vi "Apply ROIs.vi"(5 "Function":T1=enum."Write-from dataset", 7 "Mode (Redraw All)":T2, 8 "error in (no error)":errorcluster, 9 "ROIs Info []":T3[](array[typedef]) {"FOV" min=1.0 max=10.0 step=1.0; "Frame Size" min=1.0 max=10.0 step=1.0; "Laser Power" min=1.0 max=10.0 step=0.10000000149011612; "Rel. Resolution" min=1.0 max=10.0 step=1.0; "POI Dwell time" min=1.0 max=10.0 step=0.10000000149011612; "Zoom" min=1.0 max=10.0 step=0.10000000149011612}) -> (0 "error out":errorcluster, 1 "Number of ROI":i32, 3 "No ROI":bool)   [LabVIEW 2020]
uses:
  Typedefs/ROI spec.ctl
  Typedefs/ROI ID Enum.ctl
  ROI Entry screen/Typedefs/Redraw ROI.ctl
  Typedefs/ROI management FG states.ctl
  ROI Entry screen/Typedefs/FGV ROI Time Ops.ctl
  Typedefs/ROI management Input cluster.ctl
  Global Variables/General Globals.vi
  <resource>/objmgr/IMAQImage.rc
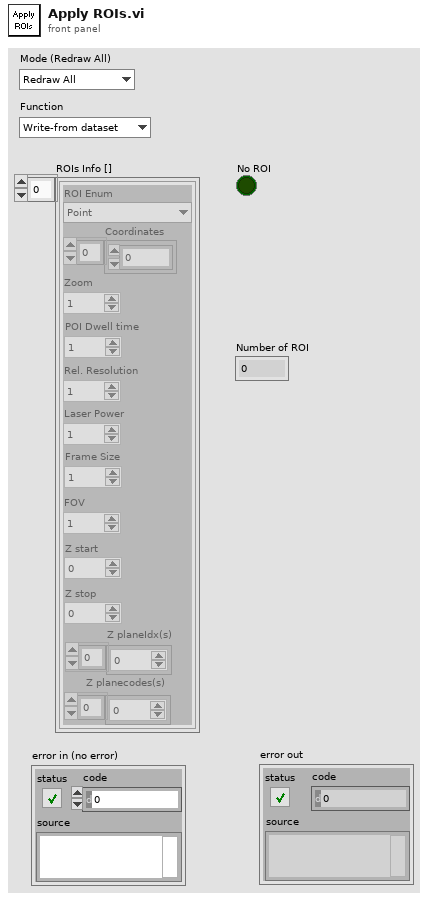
[diagram p1: front panel]
types:
  T1 = typedef "ROI management FG states.ctl" = enum16{"Read", "Write", "Write-from dataset", "Clear Last", "Clear All", "Delete ROI", "Update ROIs time", "Reload last ROI set", "Modify ROI Parameters", "Offset all ROI", "Offset visible ROI", "Modify Dwell Time", "Modify Laser Power"}
  T2 = typedef "Redraw ROI.ctl" = enum16{"Redraw All", "Redraw Deselected", "Draw Last", "Redraw Selected"}
  T3 = typedef "ROI spec.ctl" = cluster{"ROI Enum":T4, "Coordinates":i32[], "Zoom":dbl, "POI Dwell time":dbl, "Rel. Resolution":dbl, "Laser Power":dbl, "Frame Size":dbl, "FOV":dbl, "Z start":dbl, "Z stop":dbl, "Z planeIdx(s)":i32[], "Z planecodes(s)":u8[]}
  T4 = typedef "ROI ID Enum.ctl" = enum16{"Point", "MiniScan", "Comp. MiniScan", "Rectangle", "Comp. volume", "Arb. plane point", "None"}
  T5 = typedef "ROI parameters data type.ctl" = cluster{"ROI index":dbl, "ROI ID":dbl, "ROI Time (ns)":dbl, "Pixels in ROI":dbl, "X start":dbl, "Y start":dbl, "Z start":dbl, "X stop":dbl, "Y stop":dbl, "Z stop":dbl, "Angle (deg)":dbl, "Composite ID":dbl, "Number of lines":dbl, "Frame Size":dbl, "Zoom":dbl, "Laser Power (%)":dbl, "ROI group ID":dbl, "Resolution":dbl, "Dwell Time per pixel":dbl, "Pixels per miniscan":dbl, "Original FOV (um)":dbl, "Apparent Frame Size":dbl, "Z Plane Idx":i32[], "Z Plane codes":i32[]}
  T6 = typedef "FGV ROI Time Ops.ctl" = enum16{"Read", "Write Cycle Time", "Write Cycle Rate"}
  T7 = typedef "ROI management Input cluster.ctl" = cluster{"ROI Type":T4, "XY Coordinates":i32[], "Motor Z Planes":dbl[], "Dwell time per POI or per pixel (us)":dbl, "Frame size":i32, "Zoom":dbl, "Rel. Resolution":dbl, "FOV":dbl, "Laser Power (%)":dbl, "Z Plane codes":u8[], "Z start":dbl, "Z stop":dbl, "Z Plane Idx(s)":i32[]}
  T8 = typedef "IMAQ Image.ctl" = refnum<image>
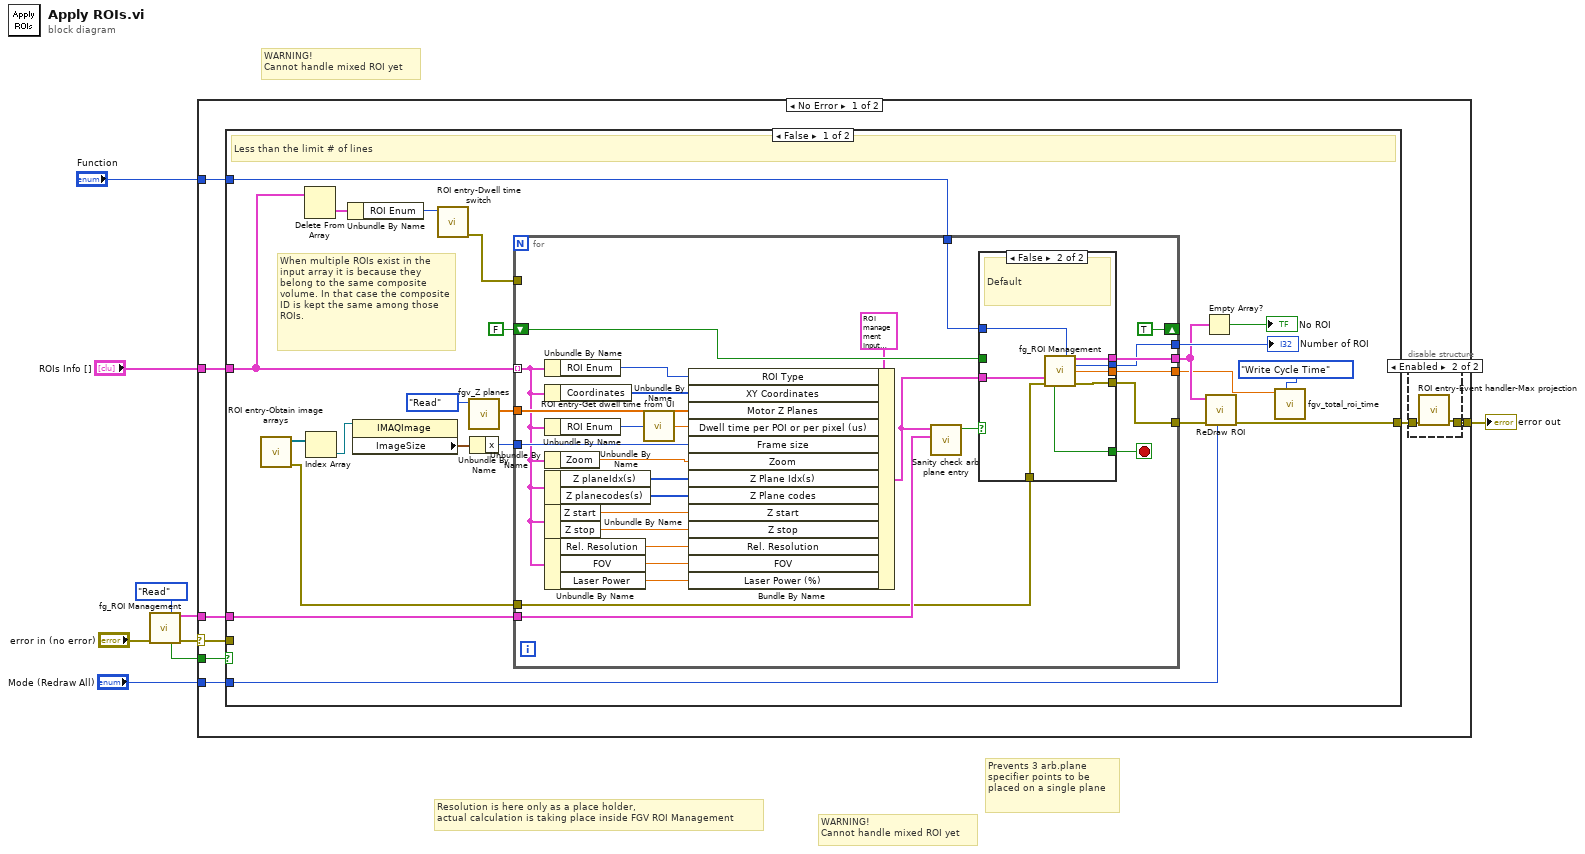
[diagram p0: block diagram]
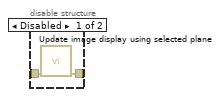
[diagram p2: hidden frame]
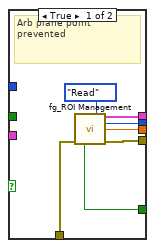
[diagram p3: hidden frame]
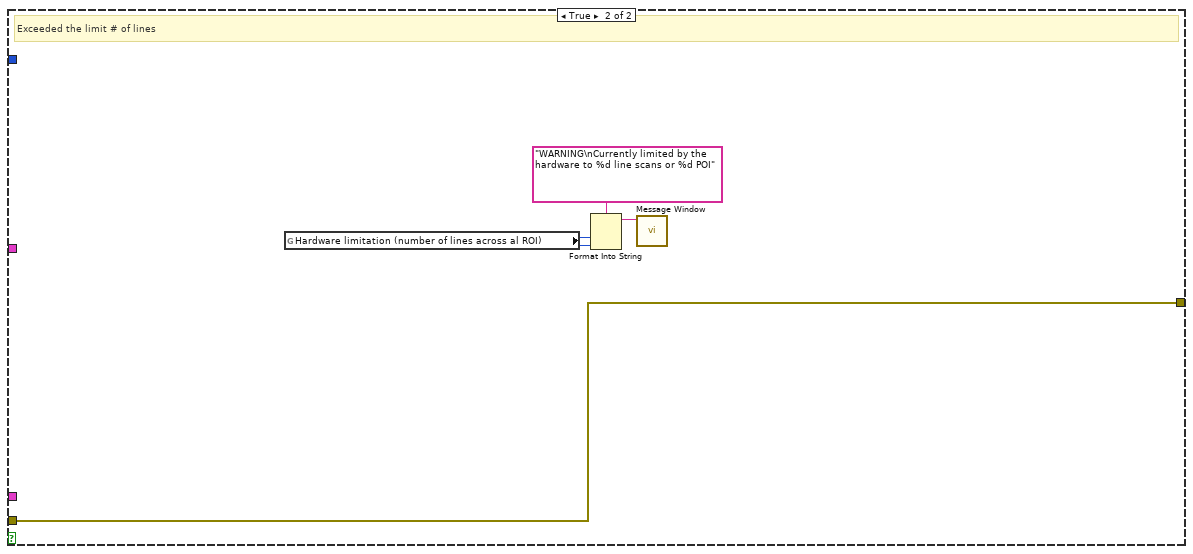
[diagram p4: hidden frame]
diagram:
  # "Resolution is here only as a place holder,\nactual calculation is taking place inside FGV ROI Management"
  # "WARNING!\nCannot handle mixed ROI yet"
  # "WARNING!\nCannot handle mixed ROI yet"
  # "Prevents 3 arb.plane specifier points to be placed on a single plane"
  n1 = call "fg_ROI Management.vi"("Function"=ROI_management_FG_states."Read", "error in (no error)"="error in (no error)") -> ("ROI Setup"=w6:T5[], "No lines left"=w1:bool, "error out"=w5:errorcluster)  [unwired: 7 in, 4 out]
  n2 = case shown="No Error" w5 {
    selector: w5 -> [w15 w91]
    tunnel: w6 -> [w17 _]
    tunnel: [w13 w91] -> w4
    tunnel: "ROIs Info []" -> [w16 _]
    tunnel: "Mode (Redraw All)" -> [w12 _]
    tunnel: "Function" -> [w11 _]
    tunnel: w1 -> [w10 _]
    frame No Error {
      n3 = case shown="False" w10 {
        tunnel: w17 -> [w38 _]
        tunnel: w16 -> [w28 _]
        tunnel: [w34 w90] -> w14
        tunnel: w15 -> [_ w90]
        tunnel: w12 -> [w29 _]
        tunnel: w11 -> [w24 _]
        frame False {
          # "When multiple ROIs exist in the input array it is because they belong to the same composite volume. In that case the composite ID is kept the same among those ROIs."
          # "Less than the limit # of lines"
          n4 = call "ROI entry-Obtain image arrays.vi"() -> ("error IO"=w33:errorcluster, "RedImageArray"=w37:T8[])  [unwired: 10 in]
          n5 = Delete From Array(array=w28) -> (deleted portion=w27:T3)  [unwired: 2 in, 1 out]
          n6 = Index Array(array=w37) -> (element=w42:T8)  [unwired: 1 in]
          n7 = Unbundle By Name(w27) -> ("ROI Enum"=w26:T4)
          n8 = property class="IMAQImage"(reference=w42) -> ("ImageSize"=w41:cluster{"x":i32, "y":i32})  [unwired: 1 in, 2 out]
          n9 = call "ROI entry-Dwell time switch.vi"("ROI Enum"=w26) -> ("error out"=w25:errorcluster)  [unwired: 10 in]
          n10 = call "fgv_Z planes.vi"("Function"=enum16{"Intialize", "Write", "Read", "Clear"}."Read") -> ("AOL Z Planes"=w35:dbl[])  [unwired: 8 in, 2 out]
          n11 = Unbundle By Name(w41) -> ("x"=w40:i32)
          n12 = for {
            tunnel: [w71] -> w31
            tunnel: w28 -> [w47] mode=indexing
            tunnel: w35 -> [w67]
            shift-right: [TRUE] -> _
            shift-left: FALSE -> [w70]
            tunnel: w40 -> [w66]
            tunnel: [w62] -> w39
            tunnel: w38 -> [w60]
            tunnel: w33 -> [w58]
            tunnel: [w57] -> w32
            tunnel: w25 -> [_]
            tunnel: w24 -> [w49]
            tunnel: [w44] -> w23
            stop <- w63 stop-if-true
            n13 = Unbundle By Name(w47) -> ("ROI Enum"=w56:T4)
            n14 = Unbundle By Name(w47) -> ("Coordinates"=w65:i32[])
            n15 = Unbundle By Name(w47) -> ("ROI Enum"=w54:T4)
            n16 = Unbundle By Name(w47) -> ("Zoom"=w64:dbl)
            n17 = Unbundle By Name(w47) -> ("Z planeIdx(s)"=w53:i32[], "Z planecodes(s)"=w52:u8[])
            n18 = Unbundle By Name(w47) -> ("Z start"=w51:dbl, "Z stop"=w50:dbl)
            n19 = Unbundle By Name(w47) -> ("Rel. Resolution"=w48:dbl, "FOV"=w46:dbl, "Laser Power"=w45:dbl)
            n20 = call "ROI entry-Get dwell time from UI.vi"("ROI Enum"=w54) -> ("Dynamic dwell time(us)"=w55:dbl)
            n21 = Bundle By Name(cluster=T7 {"ROI Type"=enum."Point", "XY Coordinates"=[], "Motor Z Planes"=[], "Dwell time per POI or per pixel (us)"=0.0, "Frame size"=0, "Zoom"=0.0, "Rel. Resolution"=0.0, "FOV"=0.0, "Laser Power (%)"=0.0, "Z Plane codes"=[], "Z start"=0.0, "Z stop"=0.0, "Z Plane Idx(s)"=[]} ("ROI management Input cluster"), "ROI Type"=w56, "XY Coordinates"=w65, "Motor Z Planes"=w67, "Dwell time per POI or per pixel (us)"=w55, "Frame size"=w66, "Zoom"=w64, "Z Plane Idx(s)"=w53, "Z Plane codes"=w52, "Z start"=w51, "Z stop"=w50, "Rel. Resolution"=w48, "FOV"=w46, "Laser Power (%)"=w45) -> (w61:T7)
            n22 = call "Sanity check arb plane entry.vi"("ROI Setup"=w60, "ROI management Input cluster"=w61) -> ("Prevent new POI"=w59:bool)  [unwired: 9 in]
            n23 = case shown="False" w59 {
              tunnel: [w78 w86] -> w71
              tunnel: w70 -> [_ _]
              tunnel: [w77 w85] -> w63
              tunnel: [w75 w84] -> w62
              tunnel: w61 -> [_ w83]
              tunnel: w58 -> [w74 w82]
              tunnel: [w73 w81] -> w57
              tunnel: w49 -> [_ w80]
              tunnel: [w72 w79] -> w44
              frame True {
                # "Arb plane point prevented"
                n24 = call "fg_ROI Management.vi"("Function"=ROI_management_FG_states."Read", "error in (no error)"=w74) -> ("ROI Setup"=w78:T5[], "Number of ROI"=w75:i32, "Total ROI time"=w72:dbl, "Exceeded limit number of lines"=w77:bool, "error out"=w73:errorcluster)  [unwired: 7 in, 2 out]
              }
              frame False {
                # "Default"
                n25 = call "fg_ROI Management.vi"("Function"=w80, "ROI management Input cluster"=w83, "error in (no error)"=w82) -> ("ROI Setup"=w86:T5[], "Number of ROI"=w84:i32, "Total ROI time"=w79:dbl, "Exceeded limit number of lines"=w85:bool, "error out"=w81:errorcluster)  [unwired: 6 in, 2 out]
              }
            }
          }
          "Number of ROI" <- w39
          n26 = Empty Array?(array=w31) -> (empty?=→"No ROI":bool)
          n27 = call "ReDraw ROI.vi"("Mode (Redraw All)"=w29, "error in"=w32, "XYZ Coordinates"=w31) -> ("error out"=w34:errorcluster)  [unwired: 8 in]
          n28 = call "fgv_total_roi_time.vi"("Op"=FGV_ROI_Time_Ops."Write Cycle Time", "Total cycle time"=w23) -> ()  [unwired: 5 in, 5 out]
        }
        frame True {
          # "Exceeded the limit # of lines"
          n29 = global read "General Globals.vi" "Hardware limitation (number of lines across al ROI)"() -> (w87:i32)
          n30 = Format Into String(format string="WARNING\nCurrently limited by the hardware to %d line scans or %d POI" ("Message string"), w87, w87) -> (resulting string=w88:string)  [unwired: 2 in, 1 out]
          n31 = call "Message Window.vi"("Message string"=w88) -> ()  [unwired: 10 in, 1 out]
        }
      }
      n32 = disable-structure shown="Enabled" {
        disable-tunnel: w14 -> [w19 w21]
        disable-tunnel: [w18 w20] -> w13
        frame Disabled {
          n33 = call "Update image display using selected plane.vi"("error in (no error)"=w19) -> ("error out"=w18:errorcluster)  [unwired: 10 in]
        }
        frame Enabled {
          n34 = call "ROI entry-Event handler-Max projection.vi"("error in (no error)"=w21) -> ("error out"=w20:errorcluster)  [unwired: 10 in]
        }
      }
    }
    frame Error {
    }
  }
  "error out" <- w4
